vi "GetAIOConfiguration.vi"(8 "error in (no error)":errorcluster, 11 "DIO_Channel in":refnum<class "AIO_Channel.lvclass">) -> (0 "error out":errorcluster, 2 "Config":refnum<class "AIO-Configuration.lvclass">, 3 "DIO_Channel out":refnum<class "AIO_Channel.lvclass">)   [LabVIEW 2021, in "AIO-Channel.lvlib" / "AIO_Channel.lvclass"]
uses:
  AIO_Channel.lvclass
  AIO_Channel.lvclass/AIO_Channel.ctl
  AIO-Configuration_class/AIO-Configuration.lvclass
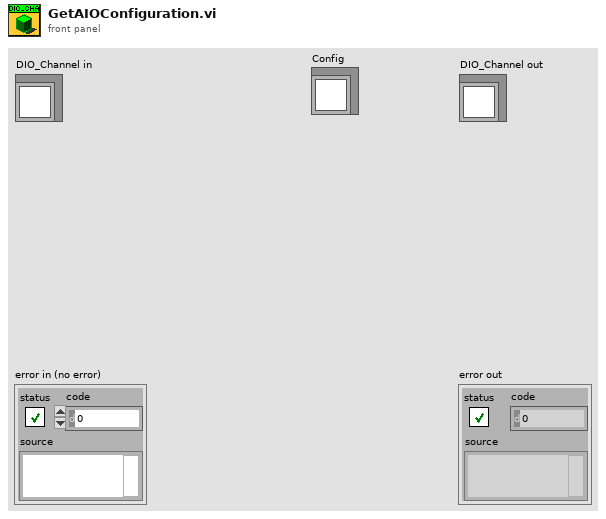
[diagram p1: front panel]
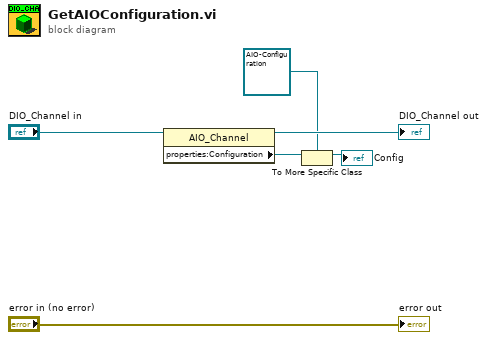
[diagram p0: block diagram]
diagram:
  n1 = property class="AIO_Channel"(reference="DIO_Channel in") -> (reference out=→"DIO_Channel out":refnum<class "AIO_Channel.lvclass">, "properties:Configuration"=w3:refnum<class "Configuration.lvclass">)  [unwired: 1 in, 1 out]
  n2 = To More Specific Class(target class=refnum<class "AIO-Configuration.lvclass"> refnum ("AIO-Channel.lvlib:DIO_CFG"), reference=w3) -> (specific class reference=→"Config":refnum<class "AIO-Configuration.lvclass">)  [unwired: 1 in, 1 out]
  "error out" <- "error in (no error)"
